vi "Load E-Series.vi"(8 "error in (no error)":errorcluster, 11 "E-Series File":path) -> (0 "error out":errorcluster, 3 "E-Series Data":T1)   [LabVIEW 2018, in "E-Series Reader.lvlib"]
doc: "Loads E-Series data from the specified <b>INI File</b>.\n\nThe VI receives the <b>E-Series File</b> path and an <b>error in</b>. It reads the E-Series file configuration and returns the loaded <b>E-Series Data</b> and the resulting <b>error out</b> status."
uses:
  E-Series Reader.lvlib
  Series Data--cluster.ctl
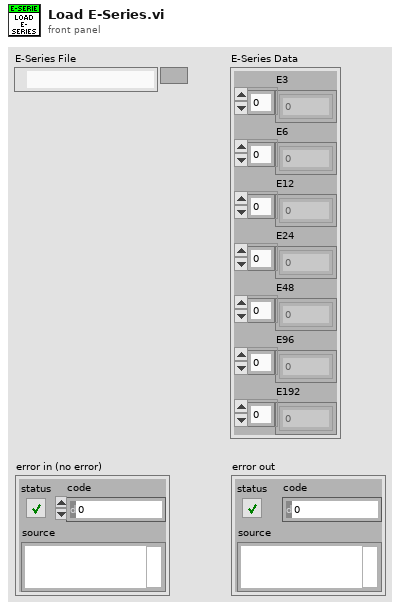
[diagram p1: front panel]
types:
  T1 = typedef "E-Series Reader.lvlib/Series Data--cluster.ctl" = cluster{"E3":u16[], "E6":u16[], "E12":u16[], "E24":u16[], "E48":u16[], "E96":u16[], "E192":u16[]}
  T2 = typedef "E-Series Reader.lvlib/E-Series File Names--array.ctl" = string[]
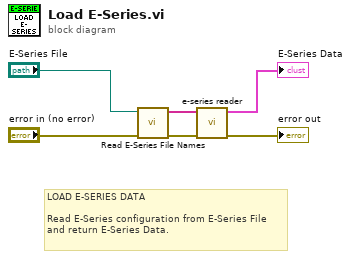
[diagram p0: block diagram]
diagram:
  # "LOAD E-SERIES DATA\n\nRead E-Series configuration from E-Series File\nand return E-Series Data."
  n1 = call "Read E-Series File Names.vi"("error in (no error)"="error in (no error)", "E-Series File"="E-Series File") -> ("error out"=w4:errorcluster, "E-Series File Names"=w3:T2)  [unwired: 8 in]
  n2 = call "e-series reader.vi"("error in"=w4, "E-Series File Names"=w3) -> ("error out"=→"error out":errorcluster, "E-Series Data"=→"E-Series Data":T1)  [unwired: 8 in]
